vi "ObserverDemo.vi"() -> ()   [LabVIEW 2017]
uses:
  Weather Station/WeatherData.lvclass
  ConsoleOut/Print Options.ctl
  Observer/Observer.lvclass
  GeneralDisplay/GeneralDisplay.lvclass
  ForecastDisplay/ForecastDisplay.lvclass
  StatisticsDisplay/StatisticsDisplay.lvclass
  CoolDisplay/CoolDisplay.lvclass
  C:/Users/fflores/Documents/LabVIEW-Open-Projects/LabIVEW OOP Design Patterns/Observer Pattern/Observer Pattern Example/Observer/Observer.lvclass
panel:
  out "error out":errorcluster
  in  "Select a Display":i32(listbox)
  in  "Stop Button":bool
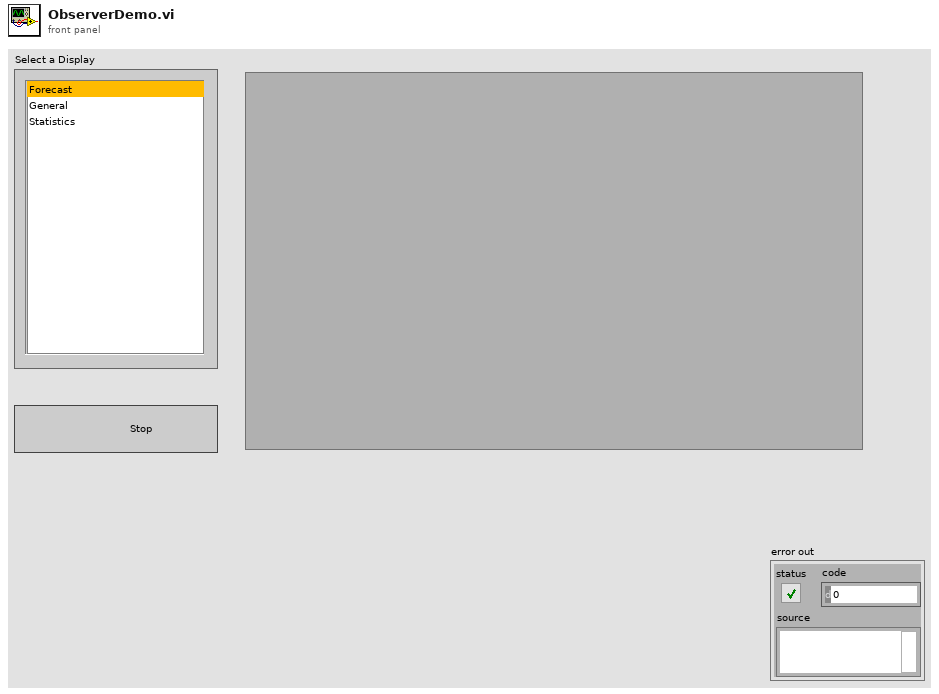
[diagram p1: front panel]
types:
  T1 = typedef "Print Options.ctl" = enum16{"Create", "Get Reference", "Print", "Print Header", "Close"}
  T2 = cluster{"Temperature":dbl, "Humidity":dbl, "Pressure":dbl, "Stop?":bool}
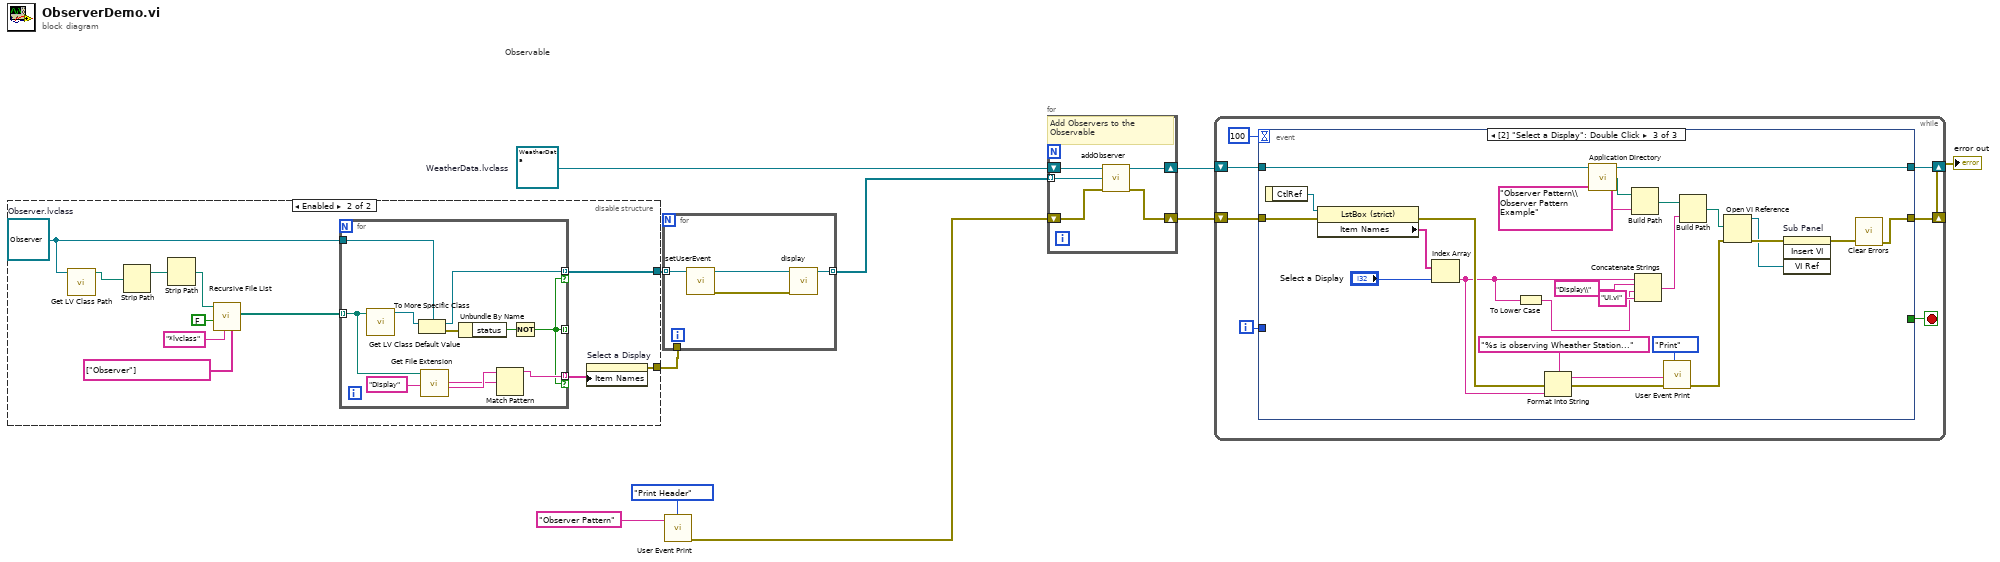
[diagram p0: block diagram]
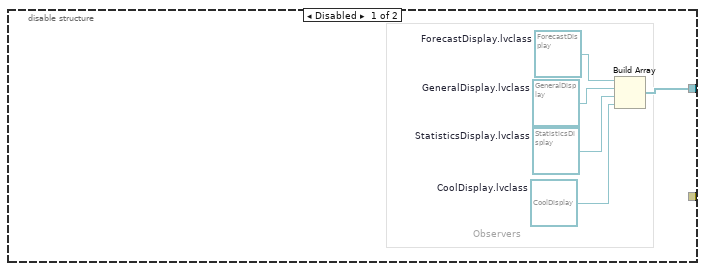
[diagram p2: hidden frame]
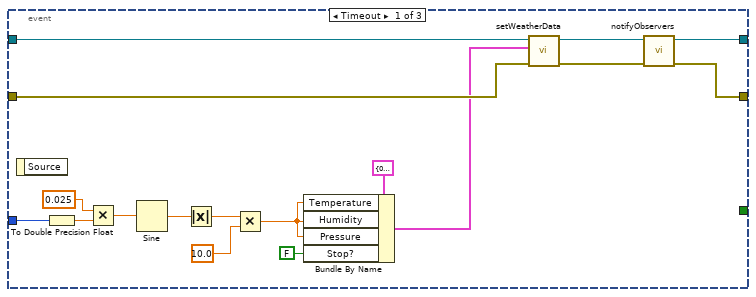
[diagram p3: hidden frame]
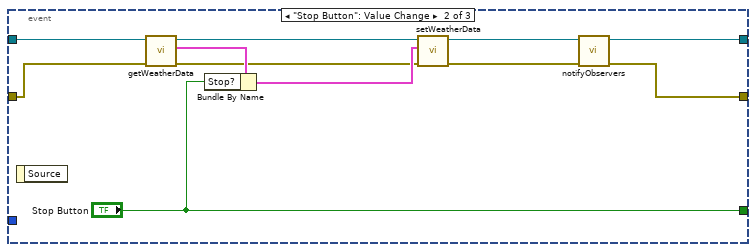
[diagram p4: hidden frame]
diagram:
  w10 = refnum<class "WeatherData.lvclass"> refnum  # WeatherData.lvclass
  # "Observable"
  n1 = disable-structure shown="Enabled" {
    disable-tunnel: [w15 w18] -> w2
    disable-tunnel: [_ w16] -> w1
    frame Disabled {
      w11 = refnum<class "CoolDisplay.lvclass"> refnum  # CoolDisplay.lvclass
      w12 = refnum<class "StatisticsDisplay.lvclass"> refnum  # StatisticsDisplay.lvclass
      w13 = refnum<class "GeneralDisplay.lvclass"> refnum  # GeneralDisplay.lvclass
      w14 = refnum<class "ForecastDisplay.lvclass"> refnum  # ForecastDisplay.lvclass
      # "Observers"
      n2 = Build Array(w14, w13, w12, w11) -> (w15:refnum<class "Observer.lvclass">[])
    }
    frame Enabled {
      w22 = refnum<class "Observer.lvclass"> refnum  # Observer.lvclass
      n3 = call <vilib>:"Get LV Class Path.vi"("object"=w22) -> ("class path"=w24:path)  [unwired: 9 in, 1 out]
      n4 = Strip Path(path=w24) -> (stripped path=w23:path)  [unwired: 1 out]
      n5 = Strip Path(path=w23) -> (stripped path=w26:path)  [unwired: 1 out]
      n6 = call <vilib>:"Recursive File List.vi"("Folders to Exclude"=string[] ["Observer"], "pattern"="*lvclass", "Continue Recursing on Error? (F)"=FALSE, "Folder Path"=w26) -> ("All Files in Dir"=w25:path[])  [unwired: 3 in, 4 out]
      n7 = for {
        tunnel: w25 -> [w32] mode=indexing
        tunnel: w22 -> [w34]
        tunnel: [w33] -> w18 mode=indexing if=w28
        tunnel: [w28] -> _ mode=indexing
        tunnel: [w29] -> w17 mode=indexing if=w28
        n8 = call <vilib>:"Get LV Class Default Value.vi"("class path"=w32) -> ("object"=w36:refnum<class>)  [unwired: 9 in, 1 out]
        n9 = To More Specific Class(target class=w34, reference=w36) -> (specific class reference=w33:refnum<class "Observer.lvclass">, error out=w27:errorcluster)  [unwired: 1 in]
        n10 = call <vilib>:"Get File Extension.vi"("file"=w32) -> ("filename without extension"=w31:string)  [unwired: 6 in, 4 out]
        n11 = Unbundle By Name(w27) -> ("status"=w35:bool)
        n12 = Match Pattern(string=w31, regular expression="Display") -> (before substring=w29:string)  [unwired: 1 in, 3 out]
        n13 = Not(x=w35) -> (.not. x?=w28:bool)
      }
      n14 = property on="Select a Display" class="LstBox (strict)"("Item Names"=w17) -> (error out=w16:errorcluster)  [unwired: 2 in, 1 out]
    }
  }
  n15 = for {
    tunnel: [w38] -> w3 mode=indexing
    tunnel: w2 -> [w37] mode=indexing
    tunnel: w1 -> [_]
    n16 = call-dynamic "setUserEvent.vi"("Observer in"=w37) -> ("error out"=w40:errorcluster, "Observer out"=w39:refnum<class "Observer.lvclass">)  [unwired: 9 in]
    n17 = call-dynamic "display.vi"("error in (no error)"=w40, "Observer in"=w39) -> ("Observer out"=w38:refnum<class "Observer.lvclass">)  [unwired: 8 in, 1 out]
  }
  n18 = call "User Event Print.vi"("Options"=Print_Options."Print Header", "String to Print"="Observer Pattern") -> ("error out"=w6:errorcluster)  [unwired: 8 in, 1 out]
  n19 = for {
    shift-right: [w44] -> w9
    shift-left: w10 -> [w45]
    shift-right: [w42] -> w5
    shift-left: w6 -> [w43]
    tunnel: w3 -> [w41] mode=indexing
    # "Add Observers to the Observable"
    n20 = call-dynamic "addObserver.vi"("error in (no error)"=w43, "Observer.lvclass"=w41, "Observable in"=w45) -> ("error out"=w42:errorcluster, "Observable out"=w44:refnum<class "WeatherData.lvclass">)  [unwired: 7 in]
  }
  n21 = while {
    shift-right: [w51] -> _
    shift-left: w9 -> [w52]
    shift-right: [w46] -> w4
    shift-left: w5 -> [w47]
    i -> [w48]
    stop <- w49 stop-if-true
    n22 = event shown="[2] \"Select a Display\": Double Click" {
      selector: _ -> [_ _ _]
      dyn-events: _ -> [_ _ _]
      timeout: 100 -> [_ _ _]
      tunnel: w52 -> [w69 w80 w104]
      tunnel: [w66 w78 w104] -> w51
      tunnel: [_ "Stop Button" _] -> w49
      tunnel: w48 -> [w63 _ _]
      tunnel: w47 -> [w56 w73 w88]
      tunnel: [w54 w70 w84] -> w46
      event Timeout {
        n23 = event-data() -> ()  [unwired: 1 in, 1 out]
        n24 = To Double Precision Float(number=w63) -> (double precision float=w62:dbl)
        n25 = Multiply(x=0.025, y=w62) -> (x*y=w61:dbl)
        n26 = Sine(x=w61) -> (sin(x)=w59:dbl)
        n27 = Absolute Value(x=w59) -> (abs(x)=w57:dbl)
        n28 = Multiply(x=w57, y=10.0) -> (x*y=w67:dbl)
        n29 = Bundle By Name(cluster=T2 {"Temperature"=0.0, "Humidity"=0.0, "Pressure"=0.0, "Stop?"=FALSE} ("WeatherData"), "Temperature"=w67, "Humidity"=w67, "Pressure"=w67, "Stop?"=FALSE) -> (w53:T2)
        n30 = call-dynamic "setWeatherData.vi"("error in (no error)"=w56, "WeatherData"=w53, "WeatherData in"=w69) -> ("error out"=w55:errorcluster, "WeatherData out"=w68:refnum<class "WeatherData.lvclass">)  [unwired: 7 in]
        n31 = call-dynamic "notifyObservers.vi"("error in (no error)"=w55, "WeatherData in"=w68) -> ("error out"=w54:errorcluster, "WeatherData out"=w66:refnum<class "WeatherData.lvclass">)  [unwired: 8 in]
      }
      event "Stop Button": Value Change {
        n32 = event-data() -> ()  [unwired: 1 in, 1 out]
        n33 = call-dynamic "getWeatherData.vi"("error in (no error)"=w73, "WeatherData in"=w80) -> ("error out"=w72:errorcluster, "WeatherData"=w75:T2, "WeatherData out"=w76:refnum<class "WeatherData.lvclass">)  [unwired: 7 in]
        n34 = Bundle By Name(cluster=w75, "Stop?"="Stop Button") -> (w77:T2)
        n35 = call-dynamic "setWeatherData.vi"("error in (no error)"=w72, "WeatherData"=w77, "WeatherData in"=w76) -> ("error out"=w71:errorcluster, "WeatherData out"=w79:refnum<class "WeatherData.lvclass">)  [unwired: 7 in]
        n36 = call-dynamic "notifyObservers.vi"("error in (no error)"=w71, "WeatherData in"=w79) -> ("error out"=w70:errorcluster, "WeatherData out"=w78:refnum<class "WeatherData.lvclass">)  [unwired: 8 in]
      }
      event "Select a Display": Double Click {
        n37 = event-data() -> ("CtlRef"=w103:refnum<vi>)  [unwired: 1 in]
        n38 = property class="LstBox (strict)"(reference=w103, error in=w88) -> (error out=w87:errorcluster, "Item Names"=w102:string[])  [unwired: 1 out]
        n39 = Index Array(array=w102, index="Select a Display") -> (element=w83:string)
        n40 = To Lower Case(string=w83) -> (all lower case string=w81:string)
        n41 = Format Into String(format string="%s is observing Wheather Station...", error in=w87, w83) -> (resulting string=w91:string, error out=w86:errorcluster)  [unwired: 1 in]
        n42 = call <vilib>:"Application Directory.vi"() -> ("Application Directory"=w100:path)
        n43 = Build Path(base path=w100, name or relative path="Observer Pattern\\Observer Pattern Example") -> (appended path=w98:path)
        n44 = Concatenate Strings(w83, "Display\\" ("string"), w81, "UI.vi" ("string")) -> (w92:string)
        n45 = call "User Event Print.vi"("Options"=Print_Options."Print", "error in (no error)"=w86, "String to Print"=w91) -> ("error out"=w85:errorcluster)  [unwired: 7 in, 1 out]
        n46 = Build Path(base path=w98, name or relative path=w92) -> (appended path=w97:path)
        n47 = Open VI Reference(vi path=w97, error in (no error)=w85) -> (vi reference=w95:refnum<vi>, error out=w96:errorcluster)  [unwired: 4 in]
        n48 = invoke on="Sub Panel" class="SubPnl" method="Insert VI"(error in=w96, "VI Ref"=w95) -> (error out=w94:errorcluster)  [unwired: 2 in, 3 out]
        n49 = call <vilib>:"Clear Errors.vi"("error in (no error)"=w94) -> ("error out"=w84:errorcluster)  [unwired: 5 in, 1 out]
      }
    }
  }
  "error out" <- w4
